vi "Set Read Notify.vi"(8 "error in (no error)":errorcluster, 9 "para1":i32, 11 "HANDLED":u32) -> (0 "error out":errorcluster)   [LabVIEW 2011, in "HID_ARZ.lvlib"]
doc: "SET_READ_NOTIFY SetReadNotify;"
uses:
  HID_ARZ.lvlib
  <userlib>/HID_ARZ/mcHID.dll
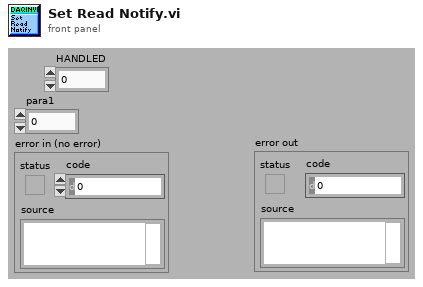
[diagram p1: front panel]
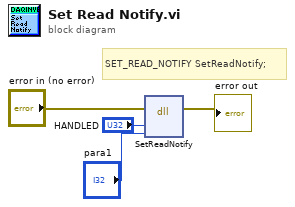
[diagram p0: block diagram]
diagram:
  # "SET_READ_NOTIFY SetReadNotify;"
  n1 = dll-call lib="C:/Program Files (x86)/National Instruments/LabVIEW 2017/user.lib/HID_ARZ/mcHID.*" fn="SetReadNotify"(error in="error in (no error)", "para0"="HANDLED", "para1"="para1") -> (error out=→"error out":errorcluster)  [unwired: 5 in, 1 out]
